vi "Execute.vi"(6 "commandTimeout":i32=-1, 7 "CommandType":i32(ring)=-1 items=["Text"=1, "StoredProcedure"=4, "TableDirect"=512], 8 "error in (no error)":errorcluster, 9 "DynamicParameters":refnum<class "DynamicParameters.lvclass">, 10 "sql":string, 11 "PGJDPMapper in":refnum<class "Mapper.lvclass">) -> (0 "error out":errorcluster, 2 "affectedRows":i32, 3 "PGJDPMapper out":refnum<class "Mapper.lvclass">)   [LabVIEW 2020, in "ORM_pgsql_jdp.lvlib" / "Mapper.lvclass"]
uses:
  Mapper.lvclass
  C:/Program Files/National Instruments/LabVIEW 2020/vi.lib/Viviota/shared/ORM.lvlibp/SqlMapper/SqlMapper.lvclass
  <vilib>/Viviota/shared/ORM.lvlibp/DynamicParameters/DynamicParameters.lvclass
  dbc/DBC.lvclass
  PGJDPParameter/Parameter.lvclass
  C:/Program Files/National Instruments/LabVIEW 2020/vi.lib/Viviota/shared/ORM.lvlibp/DynamicParameters/DynamicParameters.lvclass
  <vilib>/JDP Science/PostgreSQL Library/Connection/Execute Command (No results).vi
  <vilib>/Viviota/shared/ORM.lvlibp/SqlMapper/Read DbConnection.vi
  dbc/Read Connection.vi
  <vilib>/Viviota/shared/ORM.lvlibp/DynamicParameters/Read ParameterNames.vi
  <vilib>/Viviota/shared/ORM.lvlibp/DynamicParameters/Read ParameterValues.vi
  <vilib>/JDP Science/PostgreSQL Library/Connection/Execute Command (Result).vi
  <vilib>/JDP Science/PostgreSQL Library/Result/Clear.vi
  <vilib>/Viviota/shared/ORM.lvlibp/DbConnection/DbConnection.lvclass
  <vilib>/JDP Science/PostgreSQL Library/Connection/PQ Connection.lvclass
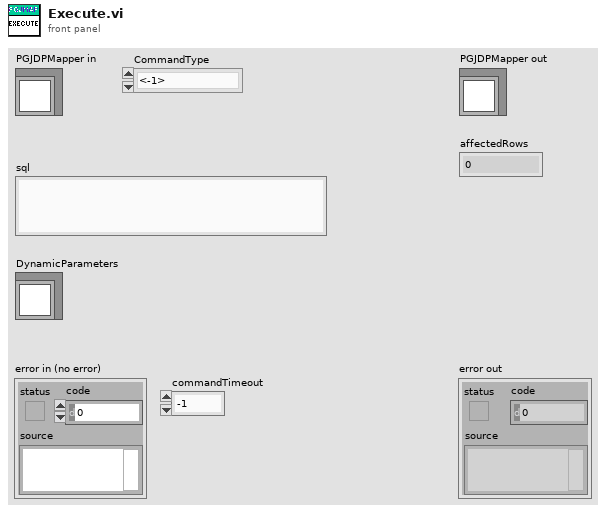
[diagram p1: front panel]
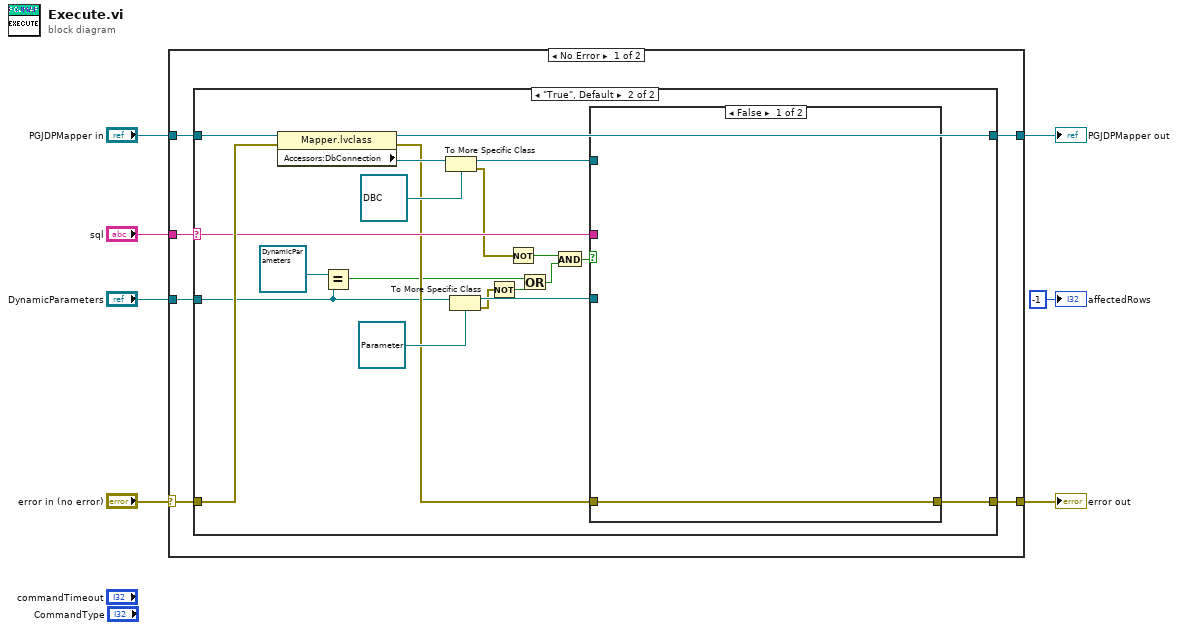
[diagram p0: block diagram]
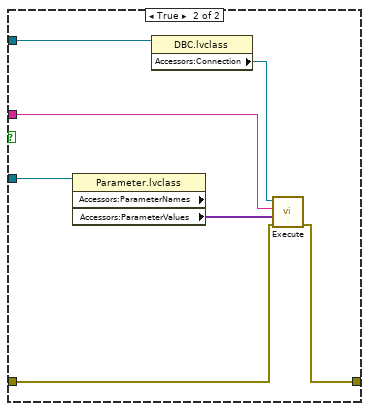
[diagram p3: hidden frame]
diagram:
  n1 = case shown="No Error" "error in (no error)" {
    selector: "error in (no error)" -> [w11 w45]
    tunnel: "PGJDPMapper in" -> [w13 w44]
    tunnel: [w12 w44] -> w6
    tunnel: [w10 w45] -> w4
    tunnel: "sql" -> [w9 _]
    tunnel: "DynamicParameters" -> [w8 _]
    frame No Error {
      n2 = case shown="\"True\", Default" w9 {
        selector: w9 -> [_ w28]
        tunnel: w13 -> [w15 w35]
        tunnel: [w15 w34] -> w12
        tunnel: w11 -> [w14 w33]
        tunnel: [w14 w25] -> w10
        tunnel: w8 -> [_ w23]
        frame "" {
        }
        frame "True", Default {
          n3 = property class="Mapper.lvclass"(reference=w35, error in=w33) -> (reference out=w34:refnum<class "Mapper.lvclass">, error out=w26:errorcluster, "Accessors:DbConnection"=w32:refnum<class "DbConnection.lvclass">)
          n4 = Equal?(x=refnum<class "DynamicParameters.lvclass"> refnum ("DynamicParameters"), y=w23) -> (x = y?=w20:bool)
          n5 = To More Specific Class(target class=refnum<class "DBC.lvclass"> refnum ("ORM_pgsql_jdp.lvlib:DBC.lvclass"), reference=w32) -> (specific class reference=w27:refnum<class "DBC.lvclass">, error out=w17:errorcluster)  [unwired: 1 in]
          n6 = To More Specific Class(target class=refnum<class "Parameter.lvclass"> refnum ("ORM_pgsql_jdp.lvlib:PGJDPParameter.lvclass"), reference=w23) -> (specific class reference=w29:refnum<class "Parameter.lvclass">, error out=w21:errorcluster)  [unwired: 1 in]
          n7 = Not(x=w21) -> (.not. x?=w22:bool)
          n8 = Not(x=w17) -> (.not. x?=w16:bool)
          n9 = Or(x=w20, y=w22) -> (x .or. y?=w18:bool)
          n10 = And(x=w16, y=w18) -> (x .and. y?=w19:bool)
          n11 = case shown="False" w19 {
            tunnel: w29 -> [_ w43]
            tunnel: w28 -> [_ w41]
            tunnel: w27 -> [_ w40]
            tunnel: w26 -> [w36 w38]
            tunnel: [w36 w37] -> w25
            frame False {
            }
            frame True {
              n12 = property class="Parameter.lvclass" props=["Accessors:ParameterNames", "Accessors:ParameterValues"](reference=w43) -> ("Accessors:ParameterValues"=w42:variant[])  [unwired: 1 in, 3 out]
              n13 = property class="DBC.lvclass"(reference=w40) -> ("Accessors:Connection"=w39:refnum<class "PQ Connection.lvclass">)  [unwired: 1 in, 2 out]
              n14 = call-poly <vilib>:"Execute.vi"("error in (no error)"=w38, "Parameters"=w42, "SQL"=w41, "PQ Connection in"=w39) -> ("error out"=w37:errorcluster)  [unwired: 6 in, 1 out]
            }
          }
        }
      }
    }
    frame Error {
    }
  }
  "error out" <- w4
  "PGJDPMapper out" <- w6
  "affectedRows" <- -1 ("affectedRows")
